vi "HexConvertion.vi"(4 "Imaging Protocol":T1, 5 "Laser(V)":dbl[](array[numeric]), 6 "Movement Correction":bool, 7 "AOL_Globals":T3={"Imaging Protocol"=enum."AOL Z-Stack", "Number of POI"=0, "Number of Miniscans"=0, "Number of Trials"=0, "Number of Cycles "=0, "# Averaged Frames"=0, "Laser power (%)"=0, "Pockels (V)"=0.0, "Acquisition Length (sec)"=0.0, "Fill time (us)"=0.0, "POI Dwell time (us)"=0.0, "Miniscan Dwell time per pixel (us)"=0.0, "PMT 1"=0.0, "PMT 2"=0.0, "Back Apperture (mA)"=200.0, "Frame Size"=0, "Center Frequency"=0.0, "Field of View (um)"=175.0, "Field of View (norm)"=0.0, "DwellTime (us)"=0.0, "Ref Dwell Time (us)"=0.0, "Wavelength (nm)"=0.0, "Zoom"=0.0, "AOL Z"=0.0, "AOL Mode"=enum."Raster", "GridXY"=0.0, "GridZ"=0.0, "TriggerPeriod (sec)"=0.0, "Number of Pixels in Miniscan"=0, "Experiment folder path"=path "", "X centre"=0.0, "Y centre"=0.0, "Angle (degrees)"=0.0, "Angle Xs (degrees)"=0.0, "Angle Ys (degrees)"=0.0, "Plane Mode"=0, "Threshold"=[], "Regenerate Chirps"=FALSE, "Rectangle ROI length (pixels)"=0, "Rectangle ROI height (pixels)"=0, "AOD fill"=4900, "StartupDelay"=0, "Samples Wait after Trigger"=5080, "Slip Cycle"=600000, "Add Cycle"=TRUE, "Functional Mode"=enum."Point", "Z Start"=0.0, "Z Stop"=0.0, "# Planes"=0, "Total Pixels"=0, "Variable Miniscan Pixels"=[], "Use Variable Length"=FALSE, "Use Variable Resolution"=FALSE, "Laser power (%) at Z Start"=0, "Laser power (%) at Z Stop"=0, "Ref Z Step"=0} {"Angle Ys (degrees)" format="%#.6g"; "Angle Xs (degrees)" format="%#.6g"; "Plane Mode" items=["XY Plane", "XZ Plane", "YZ Plane", "arbitraryplane"]; "Frame Size" items=["100X100"=100, "128X128"=128, "200X200"=200, "256X256"=256, "512X512"=512, "1024x1024"=1024, "2048x2048"=2048]; "Back Apperture (mA)" format="%#.6g"; "Pockels (V)" format="%#.6g"; "PMT 2" format="%#.6g"; "PMT 1" format="%#.6g"; "Angle (degrees)" format="%#.6g"; "POI Dwell time (us)" format="%#.6g"}, 8 "error in (no error)":errorcluster, 11 "Chirp Parameters":T2) -> (0 "error out":errorcluster, 1 "Interrupted":bool, 3 "HexPackets":string[](array[string]))   [LabVIEW 2020]
uses:
  Typedefs/Controls/AOL_Globals.ctl
  Typedefs/Imaging Protocols enum.ctl
  Typedefs/Frame Size.ctl
  Typedefs/AOL modes.ctl
  Typedefs/Plane Mode.ctl
  Typedefs/Functional Mode.ctl
  Typedefs/Chirp_ABCD.ctl
panel:
  in  "aolAmplitudes":T8={"aod1Amplitude"=210.0, "aod2Amplitude"=150.0, "aod3Amplitude"=190.0, "aod4Amplitude"=150.0}
  # "RE-ENTRANT"
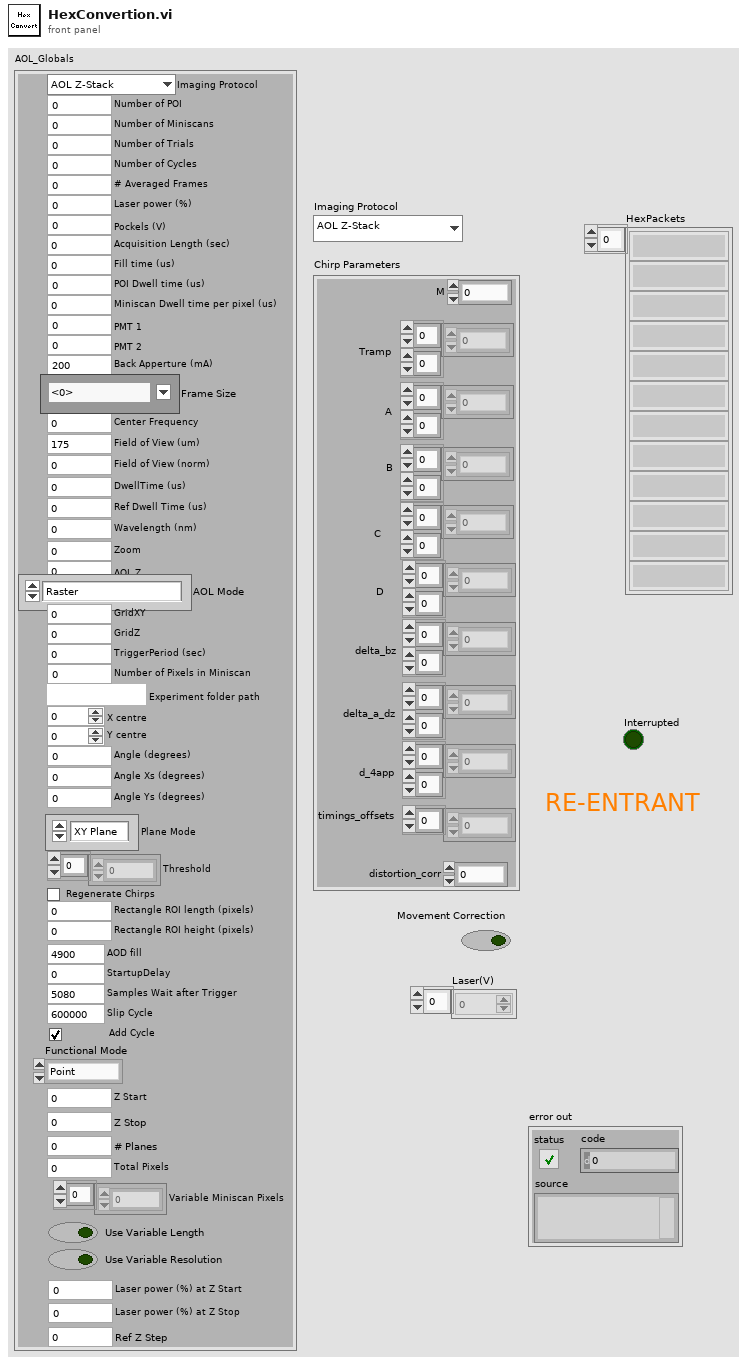
[diagram p1: front panel]
types:
  T1 = typedef "Imaging Protocols enum.ctl" = enum16{"AOL Z-Stack", "Motor Z Stack", "Parameter Sweep", "Functional Acquisition", "Single Plane Acquisition", "Volume Acquisition", "Live Imaging", "Live Plane Imaging", "Live Volume Imaging"}
  T2 = typedef "Chirp_ABCD.ctl" = cluster{"M ":dbl, "Tramp":dbl[][], "A":dbl[][], "B":dbl[][], "C":dbl[][], "D":dbl[][], "delta_bz":dbl[][], "delta_a_dz":dbl[][], "d_4app":dbl[][], "timings_offsets":dbl[], "distortion_corr":dbl}
  T3 = typedef "AOL_Globals.ctl" = cluster{"Imaging Protocol":T1, "Number of POI":u16, "Number of Miniscans":u16, "Number of Trials":u16, "Number of Cycles ":u64, "# Averaged Frames":u16, "Laser power (%)":u8, "Pockels (V)":dbl, "Acquisition Length (sec)":dbl, "Fill time (us)":dbl, "POI Dwell time (us)":dbl, "Miniscan Dwell time per pixel (us)":dbl, "PMT 1":dbl, "PMT 2":dbl, "Back Apperture (mA)":dbl, "Frame Size":T4, "Center Frequency":dbl, "Field of View (um)":dbl, "Field of View (norm)":dbl, "DwellTime (us)":dbl, "Ref Dwell Time (us)":dbl, "Wavelength (nm)":dbl, "Zoom":dbl, "AOL Z":dbl, "AOL Mode":T5, "GridXY":dbl, "GridZ":dbl, "TriggerPeriod (sec)":dbl, "Number of Pixels in Miniscan":u16, "Experiment folder path":path, "X centre":dbl, "Y centre":dbl, "Angle (degrees)":dbl, "Angle Xs (degrees)":dbl, "Angle Ys (degrees)":dbl, "Plane Mode":T6, "Threshold":u16[], "Regenerate Chirps":bool, "Rectangle ROI length (pixels)":u16, "Rectangle ROI height (pixels)":u16, "AOD fill":u16, "StartupDelay":i32, "Samples Wait after Trigger":u16, "Slip Cycle":u32, "Add Cycle":bool, "Functional Mode":T7, "Z Start":dbl, "Z Stop":dbl, "# Planes":i32, "Total Pixels":i32, "Variable Miniscan Pixels":u16[], "Use Variable Length":bool, "Use Variable Resolution":bool, "Laser power (%) at Z Start":u8, "Laser power (%) at Z Stop":u8, "Ref Z Step":i8}
  T4 = typedef "Frame Size.ctl" = u16
  T5 = typedef "AOL modes.ctl" = enum16{"Raster", "Structural", "Pointing", "Mini Scan", "Alignment"}
  T6 = typedef "Plane Mode.ctl" = u16
  T7 = typedef "Functional Mode.ctl" = enum16{"Point", "Line", "Patch", "Plane", "Volume"}
  T8 = cluster{"aod1Amplitude":dbl, "aod2Amplitude":dbl, "aod3Amplitude":dbl, "aod4Amplitude":dbl}
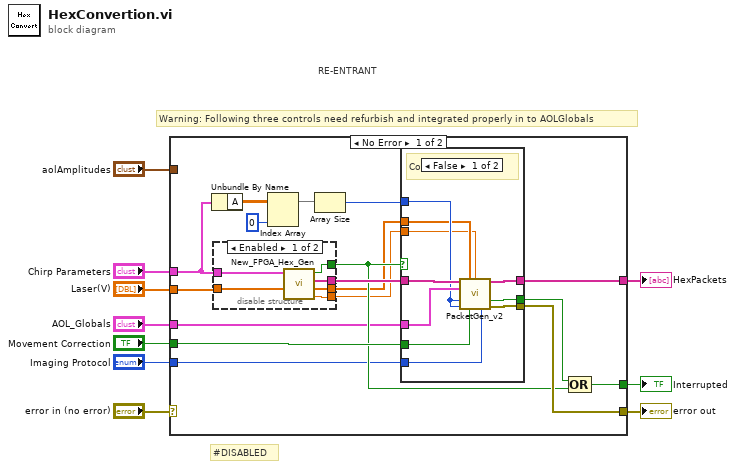
[diagram p0: block diagram]
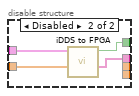
[diagram p2: hidden frame]
diagram:
  # "#DISABLED"
  # "RE-ENTRANT"
  # "Warning: Following three controls need refurbish and integrated properly in to AOLGlobals"
  n1 = case shown="No Error" "error in (no error)" {
    selector: "error in (no error)" -> [_ w48]
    tunnel: [w23 w48] -> w9
    tunnel: "aolAmplitudes" -> [_ _]
    tunnel: "AOL_Globals" -> [w13 _]
    tunnel: [w27 _] -> w6
    tunnel: "Chirp Parameters" -> [w15 _]
    tunnel: [w20 _] -> w4
    tunnel: "Movement Correction" -> [w19 _]
    tunnel: "Imaging Protocol" -> [w16 _]
    tunnel: "Laser(V)" -> [w14 _]
    frame No Error {
      n2 = Unbundle By Name(w15) -> ("A"=w26:dbl[][])
      n3 = disable-structure shown="Enabled" {
        disable-tunnel: [w30 w37] -> w22
        disable-tunnel: [w33 w34] -> w18
        disable-tunnel: w15 -> [w32 w36]
        disable-tunnel: w14 -> [w31 w35]
        disable-tunnel: [w29 _] -> w12
        disable-tunnel: [w28 _] -> w11
        frame Enabled {
          n4 = call "New_FPGA_Hex_Gen.vi"("Laser(V)"=w31, "Chirp Parameters"=w32) -> ("distortion_corr"=w28:dbl, "timings_offsets"=w29:dbl[], "HEX Array"=w30:string[], "Interrupted"=w33:bool)  [unwired: 6 in]
        }
        frame Disabled {
          n5 = call "iDDS to FPGA.vi"("Laser(V)"=w35, "Chirp Parameters"=w36) -> ("HEX Array"=w37:string[], "Interrupted"=w34:bool)  [unwired: 8 in]
        }
      }
      n6 = Index Array(array=w26, index (col)=0 ("disabled index (col)")) -> (element=w25:dbl[])  [unwired: 1 in]
      n7 = Array Size(array=w25) -> (size(s)=w17:i32)
      n8 = case shown="False" w18 {
        tunnel: w13 -> [w47 _]
        tunnel: [w46 _] -> w27
        tunnel: w17 -> [w41 _]
        tunnel: [w45 _] -> w23
        tunnel: w22 -> [w44 _]
        tunnel: [w43 _] -> w21
        tunnel: w19 -> [w42 _]
        tunnel: w16 -> [w40 _]
        tunnel: w12 -> [w39 _]
        tunnel: w11 -> [w38 _]
        frame False {
          # "Continue"
          n9 = call "PacketGen_v2.vi"("Hex Array"=w44, "timings_offsets"=w39, "distortion_corr"=w38, "AOL_Globals"=w47, "Ny"=w41, "Nx"=w41, "Movement Correction"=w42, "Imaging Protocol"=w40) -> ("HexPackets"=w46:string[], "Interrupted"=w43:bool, "error out"=w45:errorcluster)  [unwired: 4 in, 1 out]
        }
        frame True {
          # "Interrupted"
        }
      }
      n10 = Compound Arithmetic op=OR(w21, w18) -> (w20:bool)
    }
    frame Error {
    }
  }
  "error out" <- w9
  "HexPackets" <- w6
  "Interrupted" <- w4
